vi "RemoteVI Check Status Convert.vi"() -> (4 "labels":string[](array[string]), 6 "expected":string[](array[string]), 8 "actual":string[](array[string]), 10 "failures":i32)   [LabVIEW 2020]
doc: "Test support, generated by tests/caraya/build.py from tests/vectors/status.json (convert) - do not edit. Calls RemoteVI Status Convert.vi once per vector: raw and now as in the vector; the status is rendered with RemoteVI Status Text.vi and compared with the text of the vector's status. Outputs, one element per vector: labels (the vector's name), expected (rendered from the vector), actual (the VI's result rendered the same way), and failures, the number of vectors whose expected and actual differ."
uses:
  source/RemoteVI.lvlib
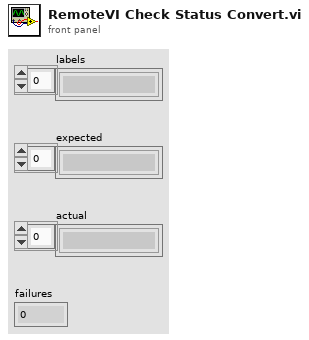
[diagram p1: front panel]
types:
  T1 = cluster{"name":string, "raw":cluster{"port":u16, "url":string, "target":string, "kind":string, "whole network":bool, "started":dbl, "updated":dbl, "clients":cluster{"address":string, "since":dbl, "last input":dbl}[], "fps":dbl, "bytes per s":dbl, "frames":u32, "latency ms":dbl, "view only":bool, "last error":string, "hWnd":u64}[], "now":dbl, "expect":string}[]
  T2 = cluster{"port":u16, "url":string, "target":string, "kind":string, "whole network":bool, "started":dbl, "updated":dbl, "clients":cluster{"address":string, "since":dbl, "last input":dbl}[], "fps":dbl, "bytes per s":dbl, "frames":u32, "latency ms":dbl, "view only":bool, "last error":string, "hWnd":u64}[]
  T3 = cluster{"port":u16, "url":string, "target":string, "kind":string, "whole network":bool, "running":bool, "uptime s":dbl, "clients":cluster{"address":string, "connected s":dbl, "idle s":dbl}[], "fps":dbl, "kB per s":dbl, "frames":u32, "latency ms":dbl, "view only":bool, "last error":string, "hWnd":u64}[]
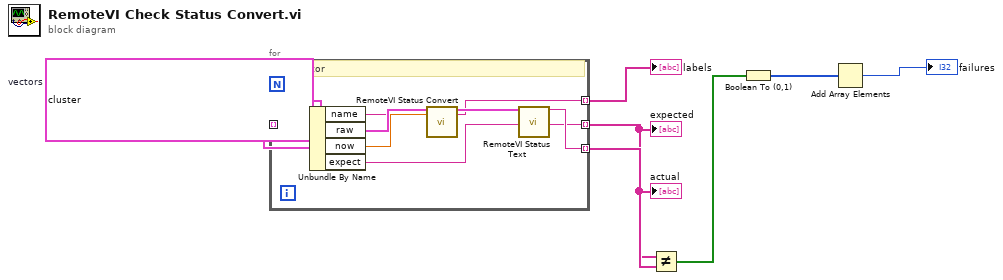
[diagram p0: block diagram]
diagram:
  w1 = T1 [{"name"="convert", "raw"=[{"port"=8088, "url"="http://127.0.0.1:8088/?t=3f9a0c1d2e4b5a6978879695a4b3c2d1", "target"="RemoteVI Demo.vi", "kind"="VI", "whole network"=FALSE, "started"=3799999934.6, "updated"=3799999999.7, "clients"=[{"address"="127.0.0.1", "since"=3799999989.8, "last input"=3799999997.3}, {"address"="192.168.1.5", "since"=3799996300.0, "last input"=0.0}], "fps"=18.04, "bytes per s"=122900.0, "frames"=1234, "latency ms"=35.2, "view only"=FALSE, "last error"="", "hWnd"=2429582}, {"port"=8100, "url"="http://pc-17:8100/?t=00ff", "target"="Untitled - Notepad", "kind"="Window", "whole network"=TRUE, "started"=3799992700.0, "updated"=3799999995.0, "clients"=[], "fps"=0.0, "bytes per s"=0.0, "frames"=0, "latency ms"=0.0, "view only"=TRUE, "last error"="TCP Write: error 66", "hWnd"=0}], "now"=3800000000.0, "expect"="Port 8088: RemoteVI Demo.vi (VI), running for 1 min 5 s, this computer only\n  http://127.0.0.1:8088/?t=3f9a0c1d2e4b5a6978879695a4b3c2d1\n  2 clients, 18.0 fps, 120 kB/s, 1234 frames, input to frame 35 ms\n  127.0.0.1, connected 10 s, last input 2 s ago\n  192.168.1.5, connected 1 h 1 min, no input yet\nPort 8100: Untitled - Notepad (Window), stopped, whole network, view only\n  http://pc-17:8100/?t=00ff\n  0 clients, 0.0 fps, 0 kB/s, 0 frames, input to frame 0 ms\n  last error: TCP Write: error 66"}]  # vectors
  n1 = for {
    tunnel: w1 -> [w8] mode=indexing
    tunnel: [w9] -> w2 mode=indexing
    tunnel: [w12] -> w3 mode=indexing
    tunnel: [w14] -> w4 mode=indexing
    # "One vector"
    n2 = Unbundle By Name(w8) -> ("name"=w9:string, "raw"=w10:T2, "now"=w11:dbl, "expect"=w12:string)
    n3 = call "RemoteVI Status Convert.vi"("raw"=w10, "now"=w11) -> ("status"=w13:T3)  [unwired: 13 in]
    n4 = call "RemoteVI Status Text.vi"("status"=w13) -> ("text"=w14:string)  [unwired: 14 in]
  }
  "labels" <- w2
  "expected" <- w3
  "actual" <- w4
  n5 = Not Equal?(x=w3, y=w4) -> (x != y?=w5:bool[])
  n6 = Boolean To (0,1)(Boolean=w5) -> (0, 1=w6:i16[])
  n7 = Add Array Elements(numeric array=w6) -> (sum=→"failures":i16)
